vi "Set Mast Position.vi"(8 "error in (no error)":errorcluster, 11 "CO3000 in":refnum<class "CO3000.lvclass">) -> (0 "error out":errorcluster, 3 "CO3000 out":refnum<class "CO3000.lvclass">)   [LabVIEW 2023, in "Turn Table and Mast.lvlib" / "CO3000.lvclass"]
uses:
  CO3000.lvclass
  CO3000.lvclass/CO3000.ctl
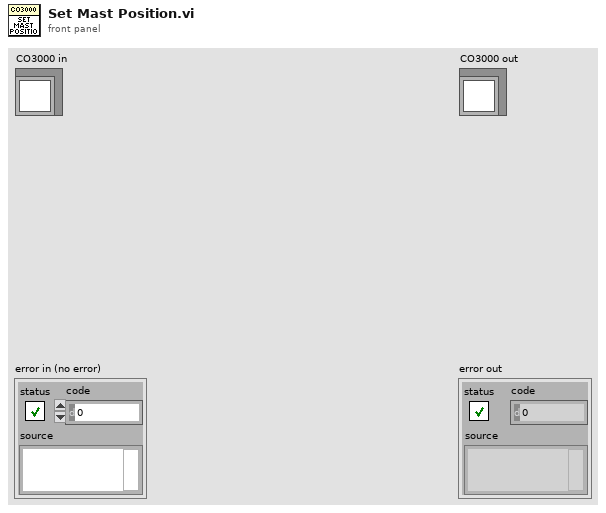
[diagram p1: front panel]
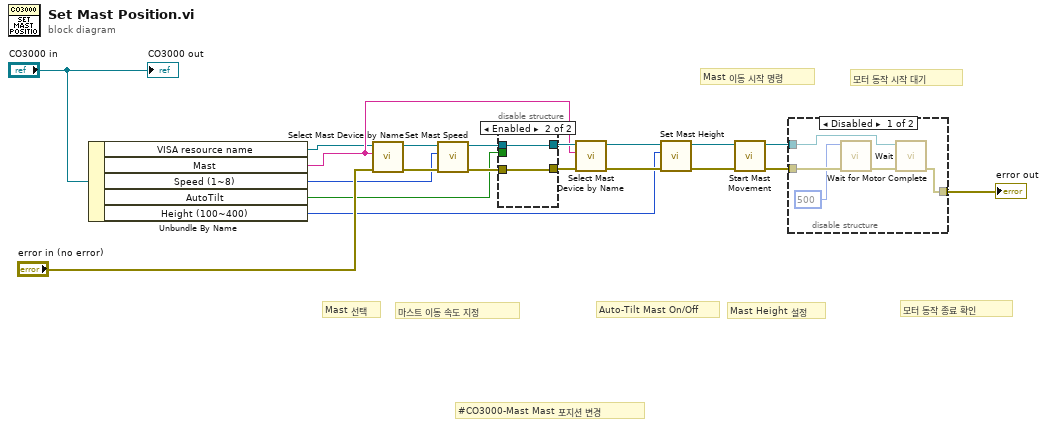
[diagram p0: block diagram]
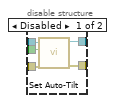
[diagram p2: hidden frame]
diagram:
  # "모터 동작 종료 확인"
  # "모터 동작 시작 대기"
  # "Mast 이동 시작 명령"
  # "Mast Height 설정"
  # "#CO3000-Mast Mast 포지션 변경"
  # "Auto-Tilt Mast On/Off"
  # "마스트 이동 속도 지정"
  # "Mast 선택"
  n1 = Unbundle By Name("CO3000 in") -> ("VISA resource name"=w2:refnum<visa-resource-name>, "Mast"=w5:string, "Speed (1~8)"=w3:i32, "AutoTilt"=w15:bool, "Height (100~400)"=w4:i32)
  n2 = call "Select Mast Device by Name.vi"("error in (no error)"="error in (no error)", "Mast Device"=w5, "VISA Refnum in"=w2) -> ("error out"=w18:errorcluster, "VISA Refnum out"=w19:refnum<visa-resource-name>)  [unwired: 7 in]
  n3 = call "Set Mast Speed.vi"("error in (no error)"=w18, "Speed (1~8)"=w3, "VISA Refnum in"=w19) -> ("error out"=w16:errorcluster, "VISA Refnum out"=w17:refnum<visa-resource-name>)  [unwired: 7 in]
  n4 = disable-structure shown="Enabled" {
    disable-tunnel: w17 -> [w25 w27]
    disable-tunnel: w16 -> [w24 w26]
    disable-tunnel: w15 -> [w23 _]
    disable-tunnel: [w22 w27] -> w9
    disable-tunnel: [w21 w26] -> w8
    frame Disabled {
      n5 = call "Set Auto-Tilt.vi"("error in (no error)"=w24, "AutoTilt"=w23, "VISA Refnum in"=w25) -> ("error out"=w21:errorcluster, "VISA Refnum out"=w22:refnum<visa-resource-name>)  [unwired: 7 in]
    }
    frame Enabled {
    }
  }
  n6 = call "Select Mast Device by Name.vi"("error in (no error)"=w8, "Mast Device"=w5, "VISA Refnum in"=w9) -> ("error out"=w7:errorcluster, "VISA Refnum out"=w6:refnum<visa-resource-name>)  [unwired: 7 in]
  n7 = call "Set Mast Height.vi"("error in (no error)"=w7, "Position (100~400)"=w4, "VISA Refnum in"=w6) -> ("error out"=w14:errorcluster, "VISA Refnum out"=w13:refnum<visa-resource-name>)  [unwired: 7 in]
  n8 = call "Start Mast Movement.vi"("error in (no error)"=w14, "VISA Refnum in"=w13) -> ("error out"=w12:errorcluster, "VISA Refnum out"=w11:refnum<visa-resource-name>)  [unwired: 8 in]
  n9 = disable-structure shown="Disabled" {
    disable-tunnel: w12 -> [w32 w33]
    disable-tunnel: w11 -> [w30 _]
    disable-tunnel: [w28 w33] -> w10
    frame Disabled {
      n10 = call "Wait.vi"("에러 상수 입력"=w32, "대기 시간 (ms)"=u32 500) -> ("에러 상수 출력"=w29:errorcluster)  [unwired: 9 in]
      n11 = call "Wait for Motor Complete.vi"("error in (no error)"=w29, "VISA Refnum in"=w30) -> ("error out"=w28:errorcluster)  [unwired: 9 in]
    }
    frame Enabled {
    }
  }
  "error out" <- w10
  "CO3000 out" <- "CO3000 in"
